vi "Map Swap Probe NI.vi"(0 "map in":map{string, dbl}(c390), 5 "key":string, 7 "value":dbl) -> (4 "map out":map{string, dbl}(c390), 6 "key already included?":bool, 8 "value unchanged?":bool)   [LabVIEW 2026]
doc: "Probe: Insert Into Map outputs map out (map) and value unchanged? (boolean)."
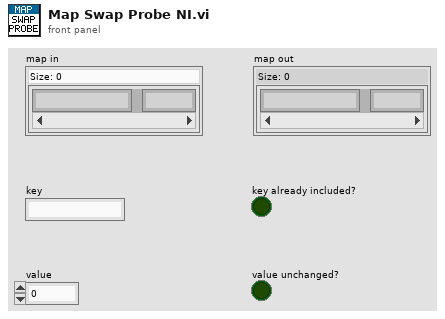
[diagram p1: front panel]
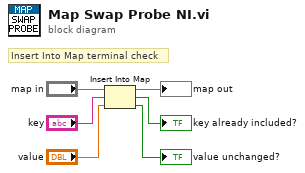
[diagram p0: block diagram]
diagram:
  # "Insert Into Map terminal check"
  n1 = Insert Into Map(map in="map in", key="key", value="value") -> (map out=→"map out":map{string, dbl}, key already included?=→"key already included?":bool, value unchanged?=→"value unchanged?":bool)
